vi "Close Transport.vi"(8 "error in":errorcluster, 11 "transport_session":T2) -> (0 "error out":errorcluster)   [LabVIEW 2015, in "Lengmur_socket.lvlib"]
uses:
  Lengmur_socket.lvlib
  Types/Transport Kind.ctl
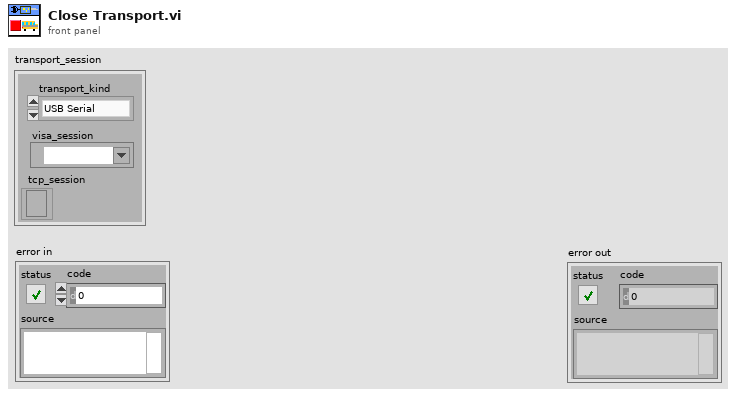
[diagram p1: front panel]
types:
  T1 = typedef "Lengmur_socket.lvlib/Transport Kind.ctl" = enum16{"USB Serial", "Ethernet TCP"}
  T2 = cluster{"transport_kind":T1, "visa_session":refnum<visa-resource-name>, "tcp_session":refnum<k5>}
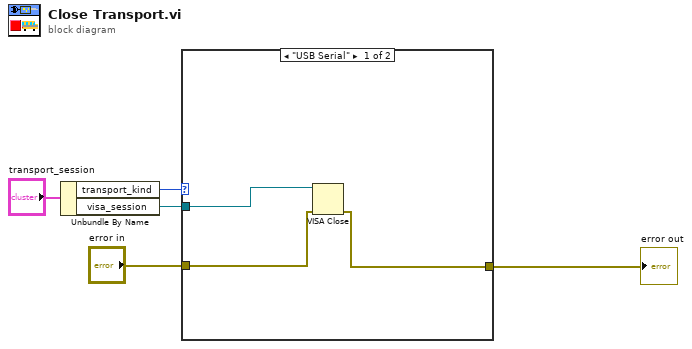
[diagram p0: block diagram]
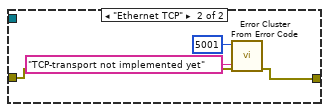
[diagram p2: hidden frame]
diagram:
  n1 = Unbundle By Name("transport_session") -> ("transport_kind"=w4:T1, "visa_session"=w3:refnum<visa-resource-name>)
  n2 = case shown="\"USB Serial\"" w4 {
    tunnel: w3 -> [w8 _]
    tunnel: "error in" -> [w7 w11]
    tunnel: [w6 w12] -> w1
    frame "USB Serial" {
      n3 = VISA Close(VISA resource name=w8, error in (no error)=w7) -> (error out=w6:errorcluster)
    }
    frame "Ethernet TCP" {
      n4 = call <vilib>:"Error Cluster From Error Code.vi"("error in (no error)"=w11, "error message (\"\")"="TCP-transport not implemented yet" ("error message (\"\")"), "error code (0)"=5001) -> ("error out"=w12:errorcluster)  [unwired: 6 in]
    }
  }
  "error out" <- w1
